vi "lvmcp_allprops.vi"() -> ()   [LabVIEW 2026]
panel:
  out "error out":errorcluster
  out "properties":T1(array[cluster])
  in  "reference":refnum<vi>
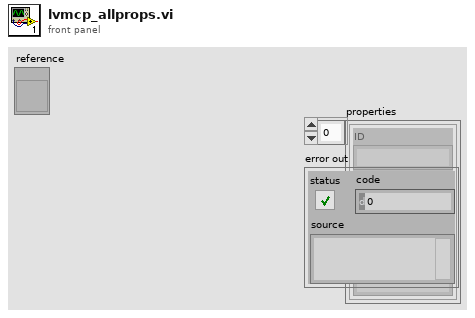
[diagram p1: front panel]
types:
  T1 = cluster{"ID":string, "Data Name":string, "Short Name":string, "Long Name":string}[]
  T2 = typedef "ASPM_ArrayOfUniqueIDStringDatanameShortnameLongname.ctl" = T3[]
  T3 = typedef "ASPM_UniqueIDStringDatanameShortnameLongname.ctl" = cluster{"Unique ID string":string, "Data name":string, "Short name (localized)":string, "Long name (localized)":string}
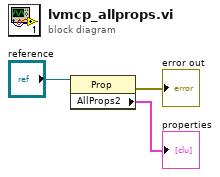
[diagram p0: block diagram]
diagram:
  n1 = property class="Prop"(reference="reference") -> (error out=→"error out":errorcluster, "AllProps2"=→"properties":T2)  [unwired: 1 in, 1 out]
